vi "TDMS_WriteBlock.vi"(8 "error in (no error)":errorcluster, 10 "Array":dbl[][](array[numeric]), 11 "Logger_state":T1={"ref TDMS"=refnum, "File Path"=path "", "counter"=0, "Folder tmp"=path "/home/lvuser/lab9data/tmp", "folder ready"=path "/home/lvuser/lab9data/ready"}) -> (0 "error out":errorcluster, 3 "state out":T1)   [LabVIEW 2025]
uses:
  Logger_State.ctl
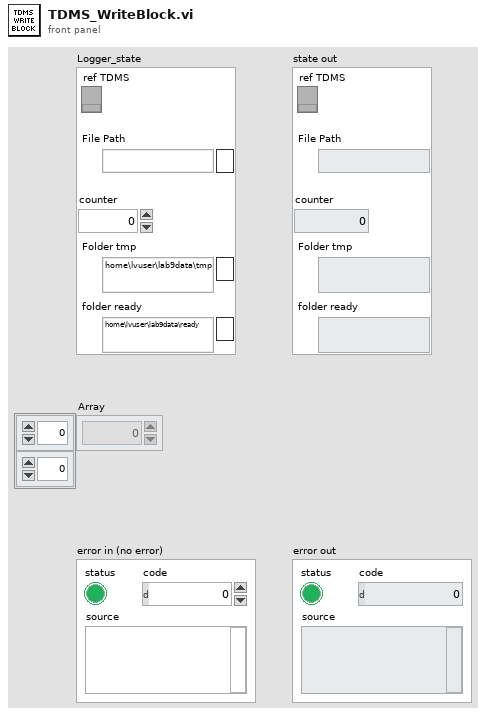
[diagram p1: front panel]
types:
  T1 = typedef "Logger_State.ctl" = cluster{"ref TDMS":refnum<k34>, "File Path":path, "counter":i32, "Folder tmp":path, "folder ready":path}
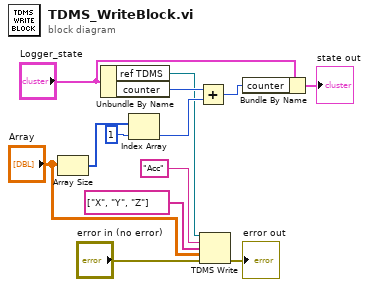
[diagram p0: block diagram]
diagram:
  n1 = Array Size(array="Array") -> (size(s)=w6:i32[])
  n2 = Unbundle By Name("Logger_state") -> ("ref TDMS"=w2:refnum<k34>, "counter"=w9:i32)
  n3 = Index Array(array=w6, index=1) -> (element=w8:i32)
  n4 = Add(x=w9, y=w8) -> (x+y=w10:i32)
  n5 = TDMS Write(0:w2, 5:"Acc" ("group name in (Untitled)"), 7:string[] ["X", "Y", "Z"] ("channel name(s) in (Untitled)"), 9:"Array", 11:"error in (no error)") -> (15:→"error out":errorcluster)  [unwired: 1 in, 3 out]
  n6 = Bundle By Name(cluster="Logger_state", "counter"=w10) -> (→"state out":T1)
